vi "filetest.vi"() -> ()   [LabVIEW 2015]
panel:
  out "All Files in Dir":path[](array[path])
  out "App:Default Data Directory":path
  out "error out":errorcluster
  in  "Path":path
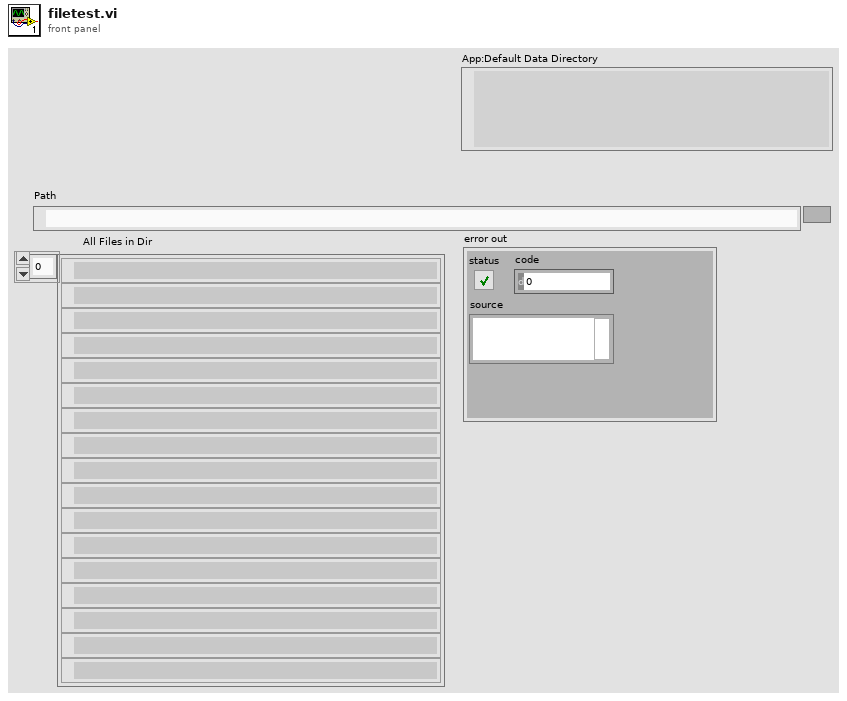
[diagram p1: front panel]
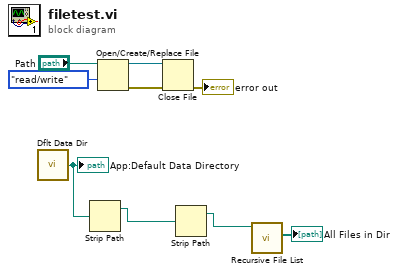
[diagram p0: block diagram]
diagram:
  n1 = call <vilib>:"Dflt Data Dir.vi"() -> ("App:Default Data Directory"=w4:path)
  "App:Default Data Directory" <- w4
  n2 = Strip Path(path=w4) -> (stripped path=w3:path)  [unwired: 1 out]
  n3 = Open/Create/Replace File(file path (use dialog)="Path", access (0:read/write)=enum16{"read/write", "read-only", "write-only"}."read/write") -> (refnum out=w9:refnum<file>, error out=w8:errorcluster)  [unwired: 4 in, 1 out]
  n4 = Close File(refnum=w9, error in=w8) -> (error out=→"error out":errorcluster)  [unwired: 1 out]
  n5 = Strip Path(path=w3) -> (stripped path=w2:path)  [unwired: 1 out]
  n6 = call <vilib>:"Recursive File List.vi"("Folder Path"=w2) -> ("All Files in Dir"=→"All Files in Dir":path[])  [unwired: 6 in, 4 out]
